vi "Calculate_DNL_INL.vi"(0 "Transition Voltage":dbl[](array[numeric]) format="%#.6g", 5 "LSB":dbl format="%#.6g", 11 "Error In":errorcluster) -> (4 "DNL":dbl[](array[numeric]) format="%#.6g", 6 "INL":dbl[](array[numeric]) format="%#.6g", 15 "Error Out":errorcluster)   [LabVIEW 2026, in "Core.lvlib"]
doc: "Calculates DNL and INL values using the supplied transition voltages and ideal LSB size."
uses:
  Core.lvlib
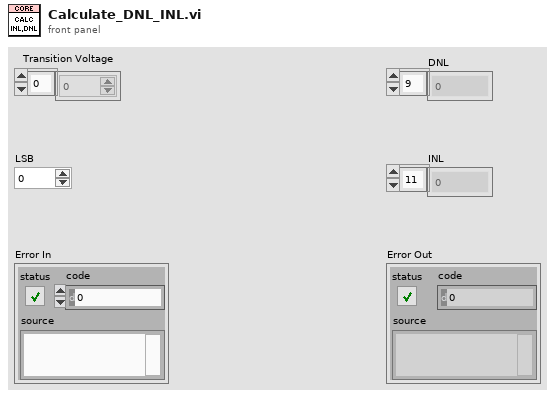
[diagram p1: front panel]
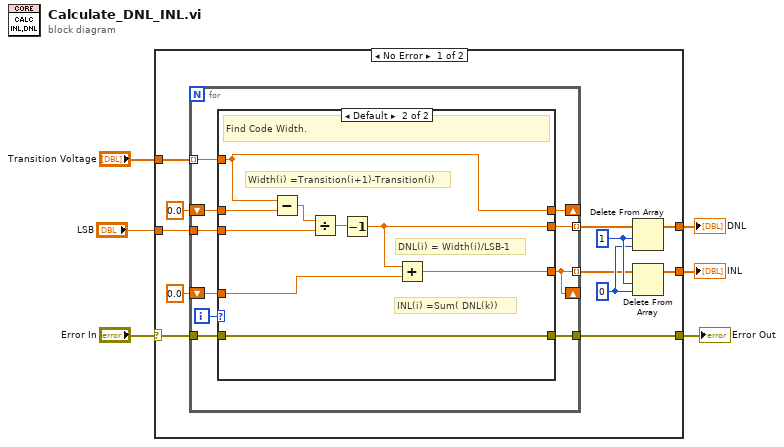
[diagram p0: block diagram]
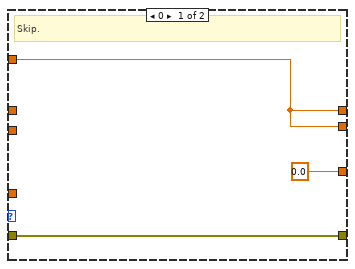
[diagram p2: hidden frame]
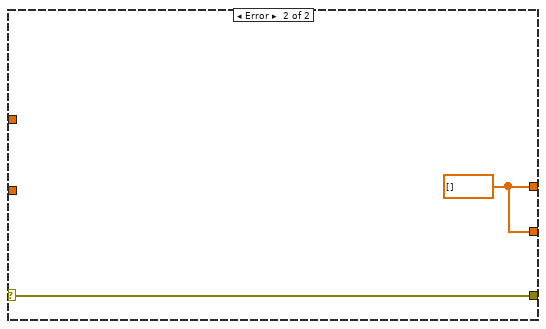
[diagram p3: hidden frame]
diagram:
  n1 = case shown="No Error" "Error In" {
    selector: "Error In" -> [w8 w41]
    tunnel: [w17 w42] -> w6
    tunnel: [w16 w42] -> w5
    tunnel: [w15 w41] -> w4
    tunnel: "LSB" -> [w10 _]
    tunnel: "Transition Voltage" -> [w7 _]
    frame No Error {
      w13 = 0 ("index")
      w14 = 1 ("length")
      n2 = for {
        tunnel: w7 -> [w26] mode=indexing
        shift-right: [w25] -> _
        shift-left: 0.0 -> [w27]
        tunnel: w8 -> [w21]
        tunnel: [w24] -> w11 mode=indexing
        tunnel: w10 -> [w23]
        tunnel: [w19] -> w12 mode=indexing
        tunnel: [w22] -> w15
        shift-right: [w19] -> _
        shift-left: 0.0 -> [w20]
        i -> [w28]
        n3 = case shown="Default" w28 {
          tunnel: w27 -> [_ w40]
          tunnel: w26 -> [w30 w39]
          tunnel: [w30 w39] -> w25
          tunnel: [w30 w34] -> w24
          tunnel: w23 -> [_ w36]
          tunnel: [0.0 w32] -> w19
          tunnel: [w29 w35] -> w22
          tunnel: w21 -> [w29 w35]
          tunnel: w20 -> [_ w33]
          frame 0 {
            # "Skip."
          }
          frame Default {
            # "INL(i) =Sum( DNL(k))"
            # "Width(i) =Transition(i+1)-Transition(i)"
            # "DNL(i) = Width(i)/LSB-1"
            # "Find Code Width."
            n4 = Subtract(x=w39, y=w40) -> (x-y=w38:dbl)
            n5 = Divide(x=w38, y=w36) -> (x/y=w37:dbl)
            n6 = Decrement(x=w37) -> (x-1=w34:dbl)
            n7 = Add(x=w34, y=w33) -> (x+y=w32:dbl)
          }
        }
      }
      n8 = Delete From Array(array=w11, length=w14, index=w13) -> (array with subset deleted=w16:dbl[])  [unwired: 1 out]
      n9 = Delete From Array(array=w12, length=w14, index=w13) -> (array with subset deleted=w17:dbl[])  [unwired: 1 out]
    }
    frame Error {
      w42 = dbl[] []
    }
  }
  "INL" <- w6
  "DNL" <- w5
  "Error Out" <- w4
